vi "Game_Step.vi"(0 "State":T1={"Tick"=0, "Phase"=0, "PhaseTicks"=0, "Level"=1, "Room"=0, "X10"=0, "Y10"=0, "VY10"=0, "Mode"=0, "Facing"=0, "Run"=0, "Vert"=0, "StandY"=0, "EntryX10"=0, "EntryY10"=0, "EntryMode"=0, "Lives"=4, "Score"=0, "NextLife"=10000, "KeyR"=0, "KeyB"=0, "KeyY"=0, "Torch"=FALSE, "FloorPhase"=0, "Dead"=FALSE, "LevelStart"=FALSE, "Quit"=FALSE, "Sound"=0, "Seed"=12345, "DemoStep"=0, "Tiles"=[], "World"=[], "Enemies"=[], "Highscores"=[], "Name"=[0, 0, 0], "Cursor"=0}, 5 "Key":u16, 7 "Rooms":T2(array[cluster]), 11 "error in":errorcluster) -> (4 "State out":T1={"Tick"=0, "Phase"=0, "PhaseTicks"=0, "Level"=1, "Room"=0, "X10"=0, "Y10"=0, "VY10"=0, "Mode"=0, "Facing"=0, "Run"=0, "Vert"=0, "StandY"=0, "EntryX10"=0, "EntryY10"=0, "EntryMode"=0, "Lives"=4, "Score"=0, "NextLife"=10000, "KeyR"=0, "KeyB"=0, "KeyY"=0, "Torch"=FALSE, "FloorPhase"=0, "Dead"=FALSE, "LevelStart"=FALSE, "Quit"=FALSE, "Sound"=0, "Seed"=12345, "DemoStep"=0, "Tiles"=[], "World"=[], "Enemies"=[], "Highscores"=[], "Name"=[0, 0, 0], "Cursor"=0}, 15 "error out":errorcluster)   [LabVIEW 2020, in "GH_Engine.lvlib"]
doc: "One game tick, a state machine over the phases Title, Ready, Playing, Paused, Dying, Treasure, LevelDone, GameOver, Name, Demo. Title: card, short instructions, then the highscore table, then the demo; Enter starts, Esc quits. Ready: short pause with a message. Playing: Game_Play; a hit or a deadly fall starts Dying, the treasure room starts Treasure. Paused: Space, Enter or an arrow continues, Esc/P again ends the game (GameOver). Dying: one life less, then Ready at the arrival point or GameOver. Treasure: playing against the clock, then LevelDone and the next level. GameOver: then Name entry (arrows choose letters, Enter saves) when the score is good enough, else Title. Sound bits for the audio loop; music during Ready, Playing, Treasure. Keys: 0 None, 1 Up, 2 Down, 3 Left, 4 Right, 5 Quit, 6 Pause, 7 Start, 8 Jump, 9 Release, 10 ReleaseV, 11 ReleaseL, 12 ReleaseR, 13 Cheat."
uses:
  GH_Engine.lvlib
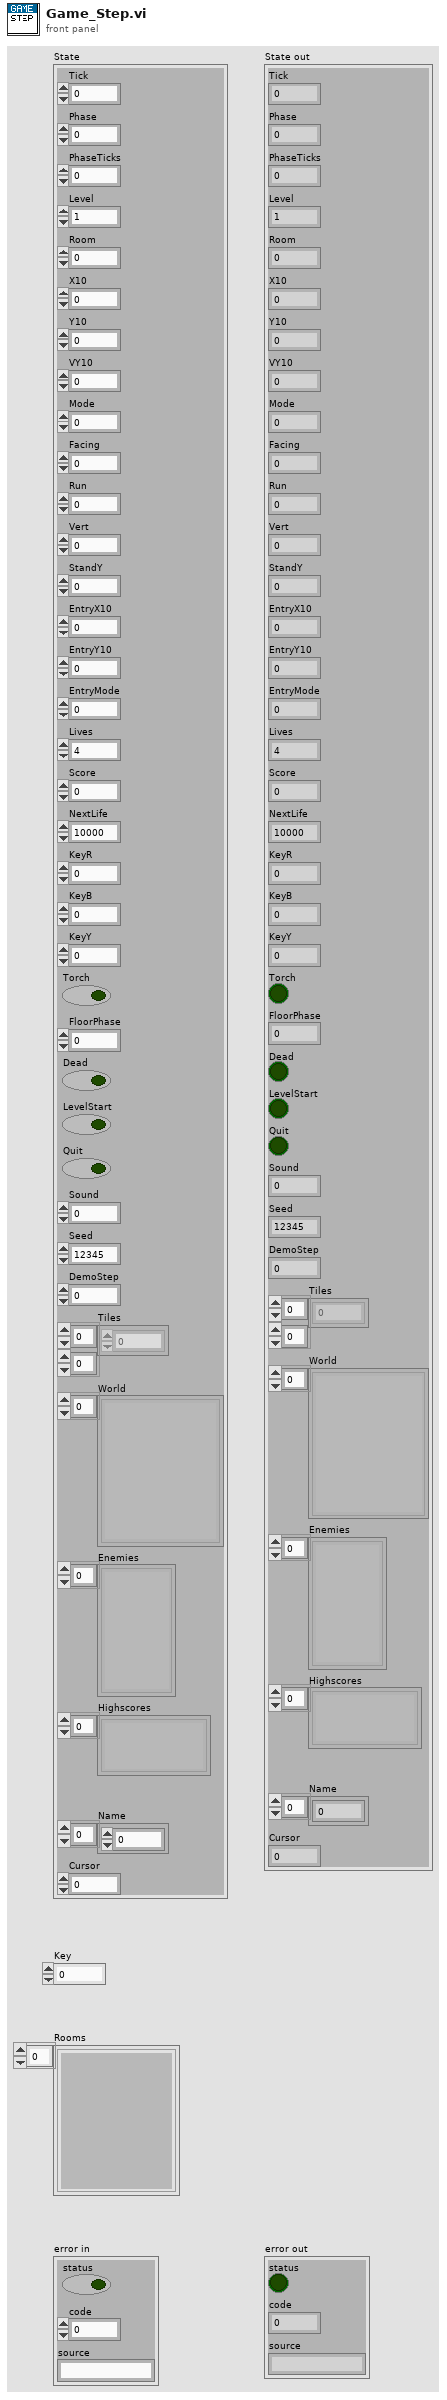
[diagram p1: front panel]
types:
  T1 = cluster{"Tick":u32, "Phase":i32, "PhaseTicks":i32, "Level":i32, "Room":i32, "X10":i32, "Y10":i32, "VY10":i32, "Mode":i32, "Facing":i32, "Run":i32, "Vert":i32, "StandY":i32, "EntryX10":i32, "EntryY10":i32, "EntryMode":i32, "Lives":i32, "Score":i32, "NextLife":i32, "KeyR":i32, "KeyB":i32, "KeyY":i32, "Torch":bool, "FloorPhase":i32, "Dead":bool, "LevelStart":bool, "Quit":bool, "Sound":i32, "Seed":u32, "DemoStep":i32, "Tiles":u8[][], "World":cluster{"ID":string, "Depth":i32, "Column":i32, "Tiles":u8[][]}[], "Enemies":cluster{"Kind":i32, "X10":i32, "Y10":i32, "Dir":i32, "Mode":i32}[], "Highscores":cluster{"Score":i32, "Name":string}[], "Name":i32[], "Cursor":i32}
  T2 = cluster{"ID":string, "Depth":i32, "Column":i32, "Tiles":u8[][]}[]
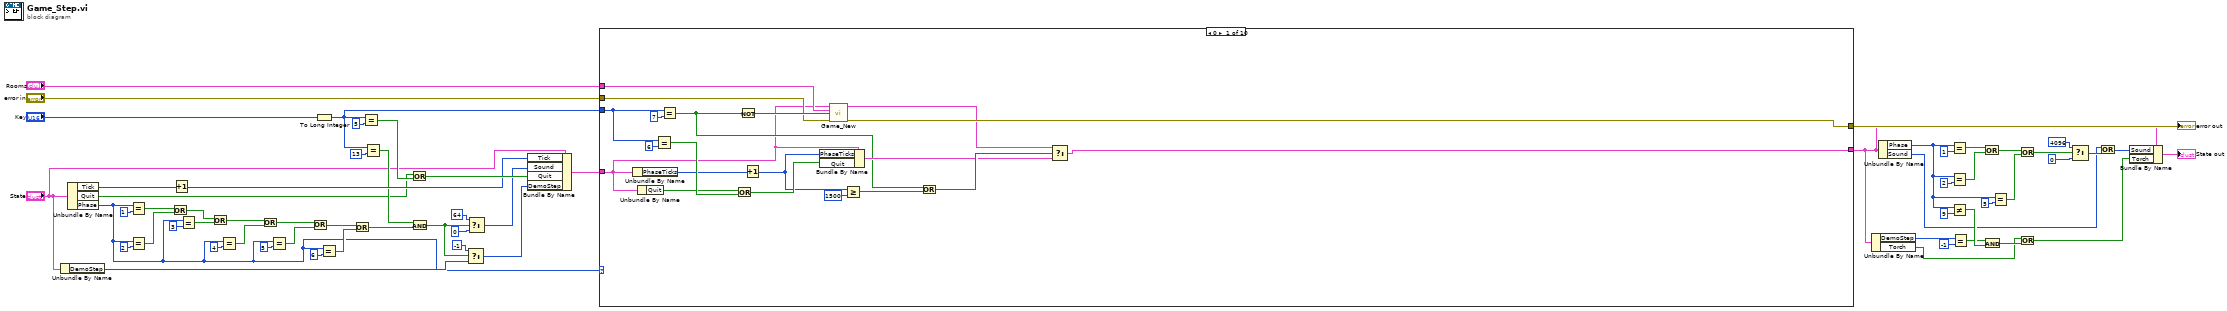
[diagram p0: block diagram]
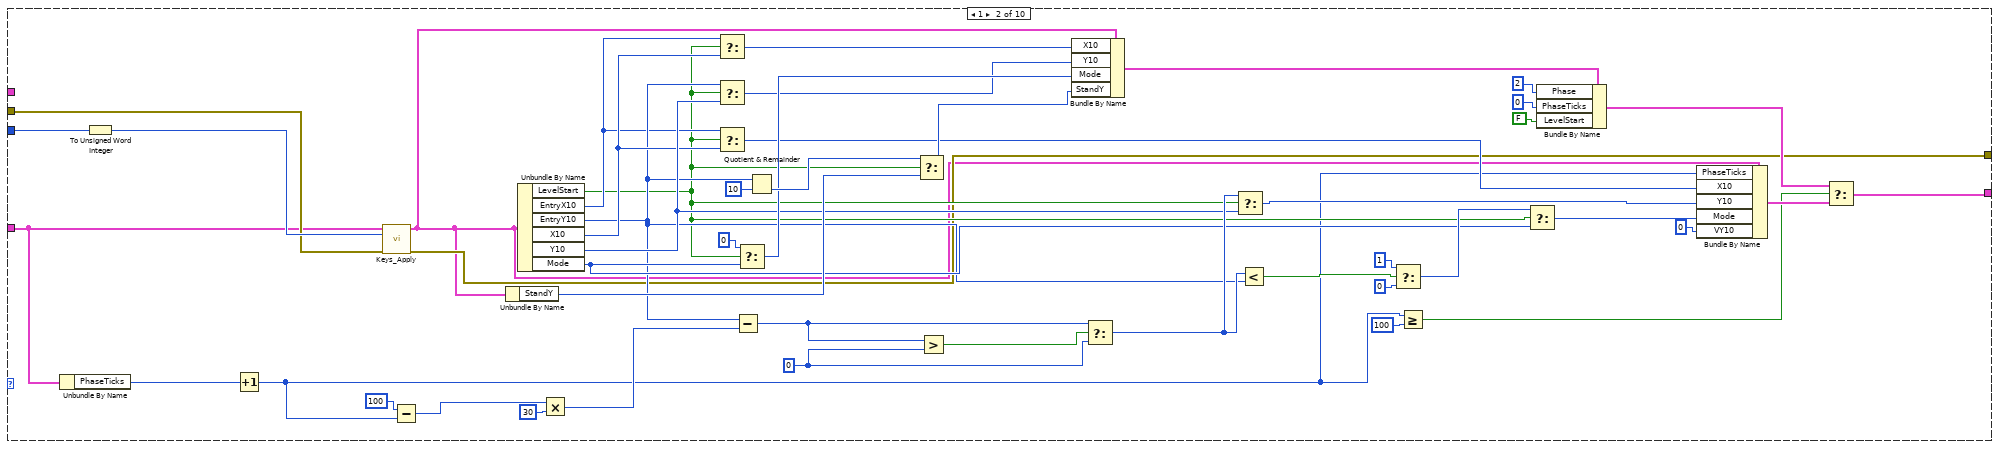
[diagram p2: hidden frame]
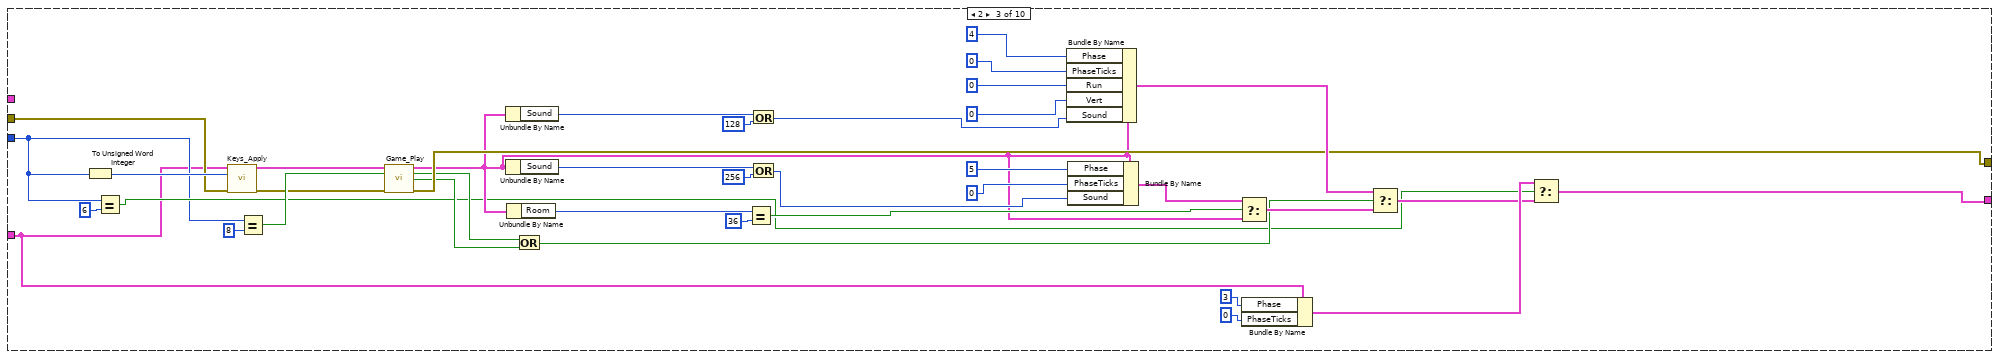
[diagram p3: hidden frame]
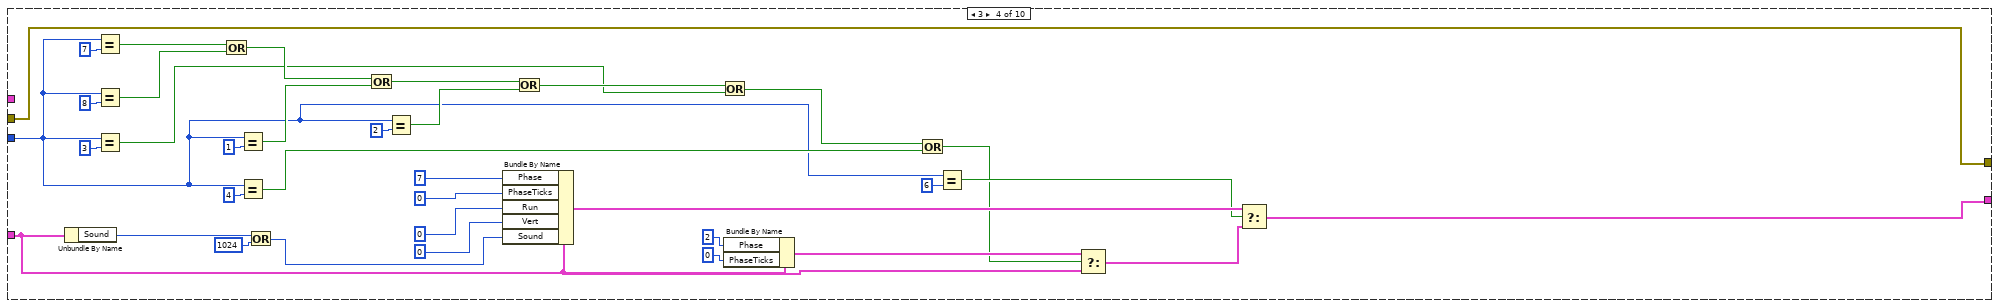
[diagram p4: hidden frame]
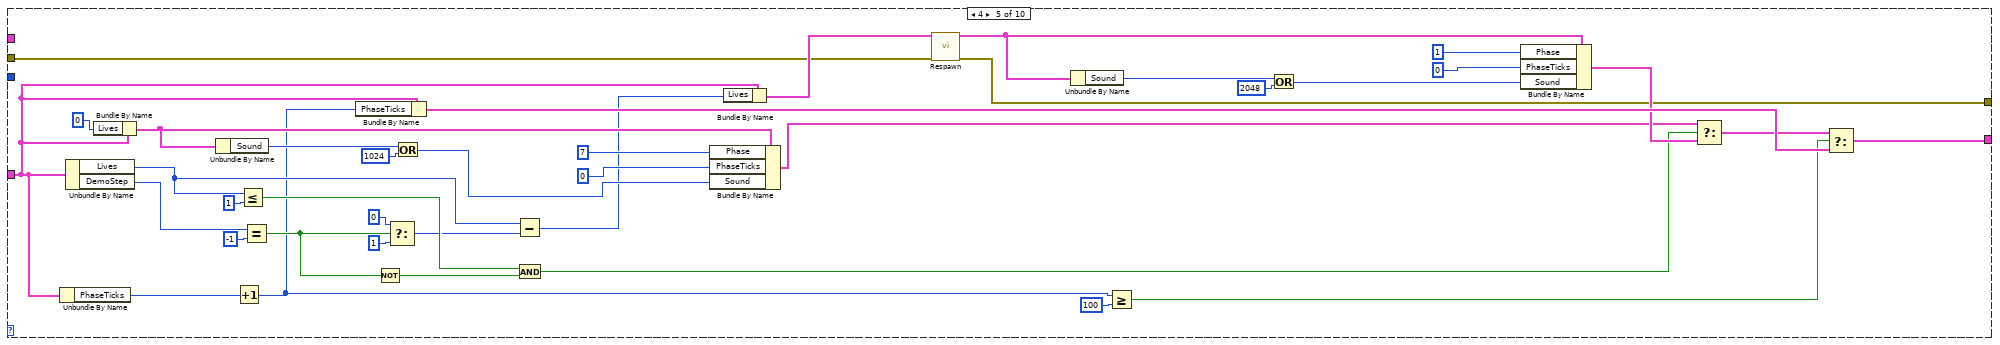
[diagram p5: hidden frame]
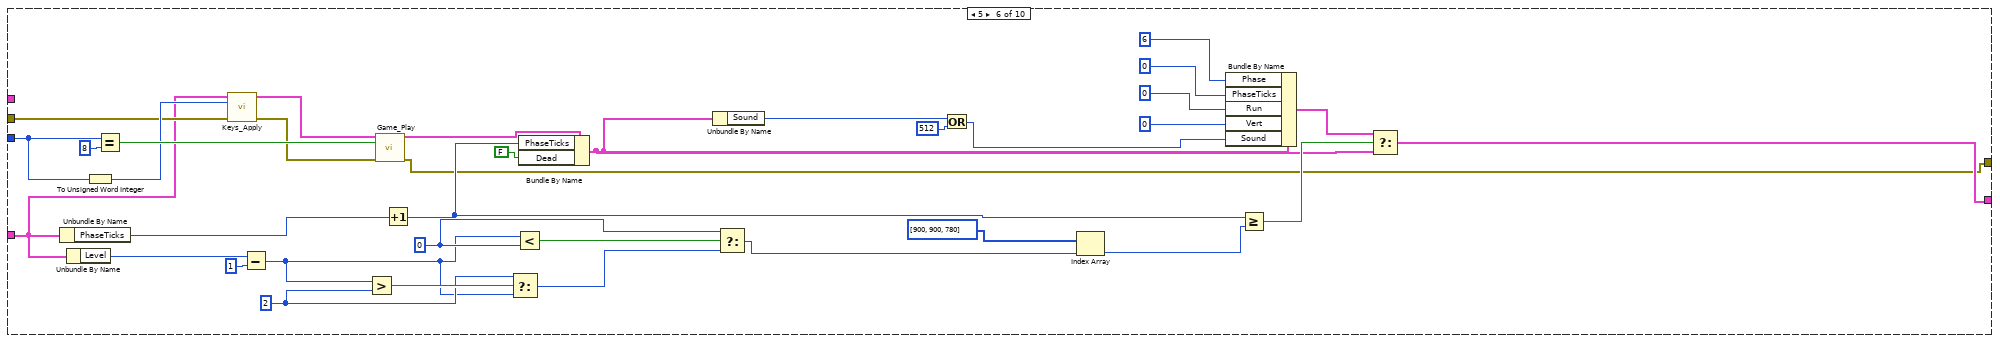
[diagram p6: hidden frame]
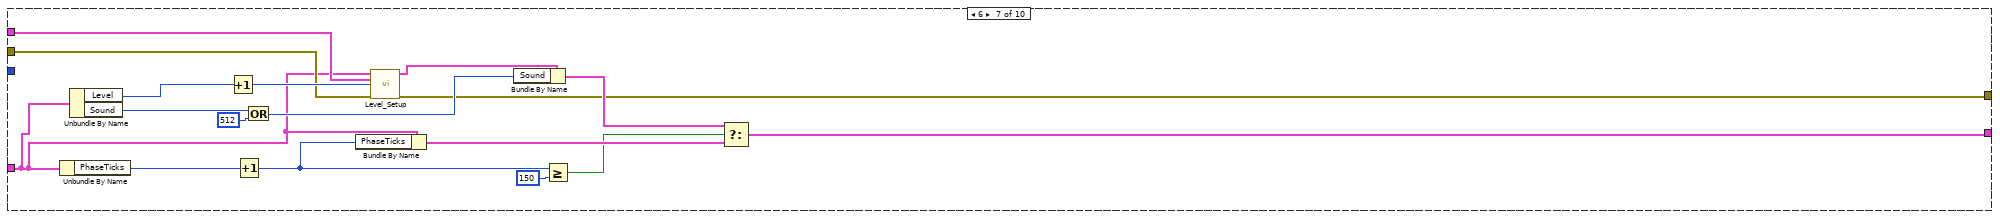
[diagram p7: hidden frame]
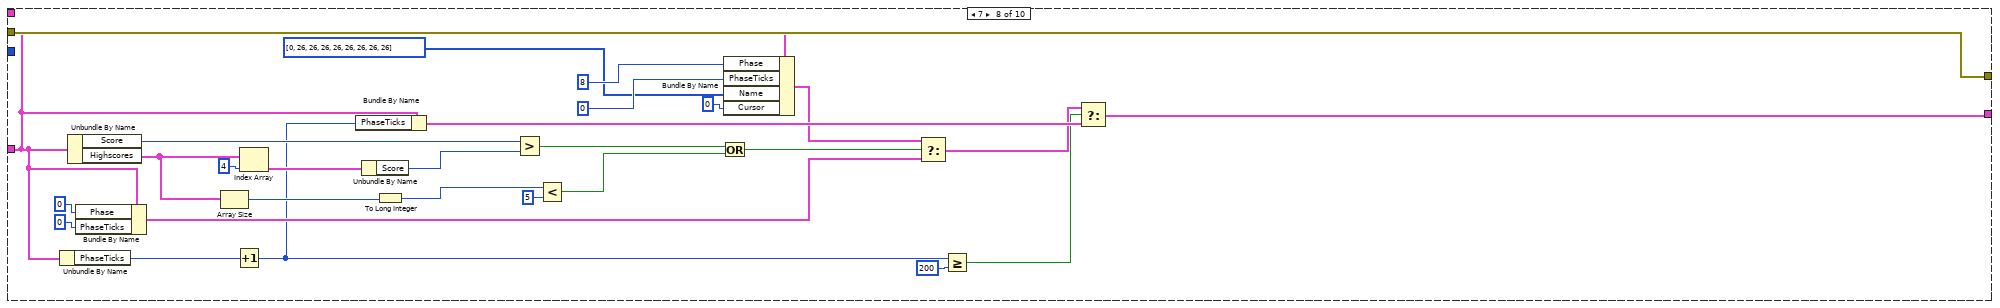
[diagram p8: hidden frame]
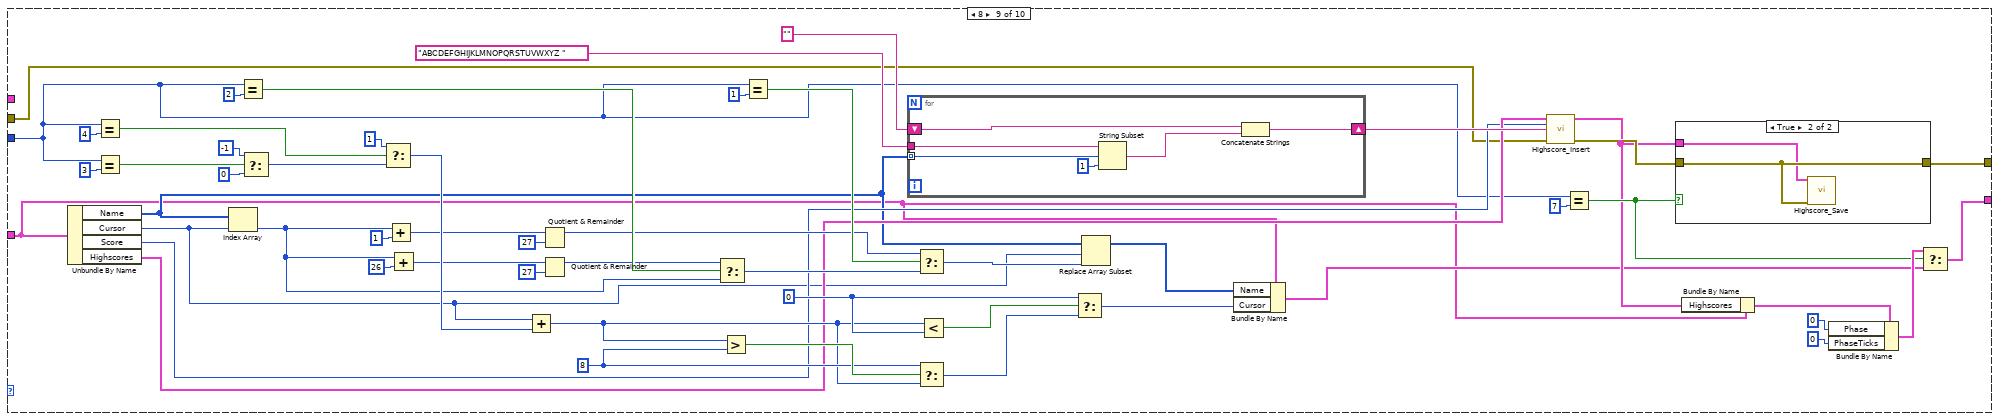
[diagram p9: hidden frame]
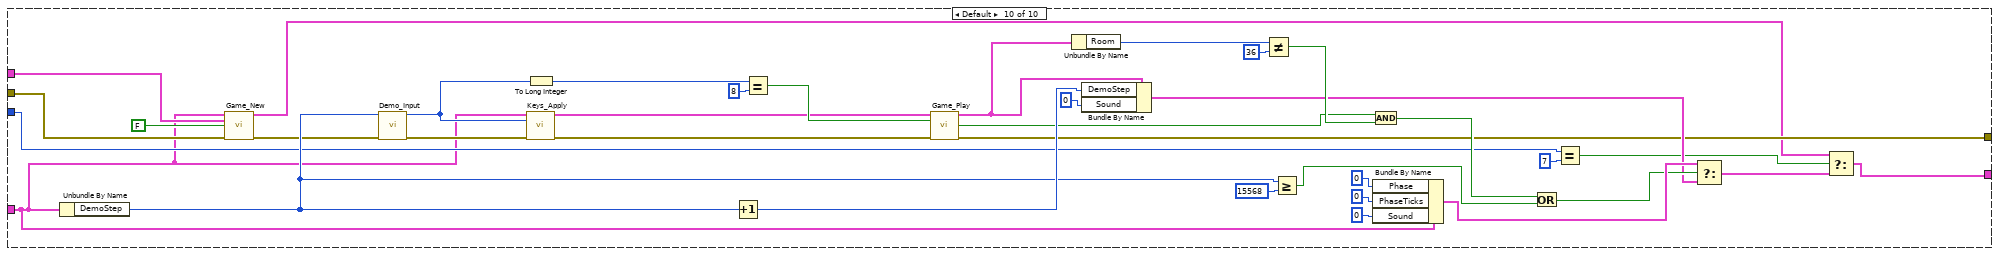
[diagram p11: hidden frame]
diagram:
  n1 = Unbundle By Name("State") -> ("DemoStep"=w29:i32)
  n2 = Unbundle By Name("State") -> ("Tick"=w6:u32, "Quit"=w7:bool, "Phase"=w8:i32)
  n3 = Equal?(x=w8, y=1) -> (x = y?=w10:bool)
  n4 = Equal?(x=w8, y=2) -> (x = y?=w12:bool)
  n5 = Or(x=w10, y=w12) -> (x .or. y?=w21:bool)
  n6 = Increment(x=w6) -> (x+1=w30:u32)
  n7 = Equal?(x=w8, y=3) -> (x = y?=w14:bool)
  n8 = Or(x=w21, y=w14) -> (x .or. y?=w22:bool)
  n9 = Equal?(x=w8, y=4) -> (x = y?=w16:bool)
  n10 = Or(x=w22, y=w16) -> (x .or. y?=w23:bool)
  n11 = Equal?(x=w8, y=5) -> (x = y?=w18:bool)
  n12 = Or(x=w23, y=w18) -> (x .or. y?=w24:bool)
  n13 = To Long Integer(number="Key") -> (32bit integer=w5:i32)
  n14 = Equal?(x=w8, y=6) -> (x = y?=w20:bool)
  n15 = Or(x=w24, y=w20) -> (x .or. y?=w25:bool)
  n16 = Equal?(x=w5, y=5) -> (x = y?=w35:bool)
  n17 = Equal?(x=w5, y=13) -> (x = y?=w27:bool)
  n18 = Or(x=w7, y=w35) -> (x .or. y?=w36:bool)
  n19 = And(x=w27, y=w25) -> (x .and. y?=w28:bool)
  n20 = Select(t=-1, s=w28, f=w29) -> (s? t:f=w38:i32)
  n21 = Select(t=64, s=w28, f=0) -> (s? t:f=w33:i32)
  n22 = Bundle By Name(cluster="State", "Tick"=w30, "Sound"=w33, "Quit"=w36, "DemoStep"=w38) -> (w39:T1)
  n23 = case shown="0" w8 {
    tunnel: "Rooms" -> [w67 _ _ _ _ _ w279 _ _ w387]
    tunnel: "error in" -> [w68 w87 w134 w172 w206 w245 w280 w296 w325 w388]
    tunnel: w5 -> [w66 w86 w133 w171 _ w244 _ _ w324 w386]
    tunnel: w39 -> [w65 w85 w132 w170 w205 w243 w278 w295 w323 w385]
    tunnel: [w77 w90 w145 w172 w219 w252 w287 w296 w370 w404] -> w41
    tunnel: [w84 w131 w169 w204 w242 w277 w294 w322 w375 w420] -> w40
    frame 0 {
      n24 = Unbundle By Name(w65) -> ("PhaseTicks"=w69:i32)
      n25 = Unbundle By Name(w65) -> ("Quit"=w78:bool)
      n26 = Equal?(x=w66, y=6) -> (x = y?=w80:bool)
      n27 = Equal?(x=w66, y=7) -> (x = y?=w72:bool)
      n28 = Or(x=w78, y=w80) -> (x .or. y?=w81:bool)
      n29 = Not(x=w72) -> (.not. x?=w75:bool)
      n30 = Increment(x=w69) -> (x+1=w70:i32)
      n31 = Bundle By Name(cluster=w65, "PhaseTicks"=w70, "Quit"=w81) -> (w82:T1)
      n32 = call "Game_New.vi"("State"=w65, "Rooms"=w67, "Demo"=w75, "error in"=w68) -> ("State out"=w76:T1, "error out"=w77:errorcluster)  [unwired: 10 in]
      n33 = Greater Or Equal?(x=w70, y=1500) -> (x >= y?=w74:bool)
      n34 = Or(x=w72, y=w74) -> (x .or. y?=w83:bool)
      n35 = Select(t=w76, s=w83, f=w82) -> (s? t:f=w84:T1)
    }
    frame 1 {
      w106 = 0
      n36 = Unbundle By Name(w85) -> ("PhaseTicks"=w91:i32)
      n37 = To Unsigned Word Integer(number=w86) -> (unsigned 16bit integer=w88:u16)
      n38 = Increment(x=w91) -> (x+1=w92:i32)
      n39 = call "Keys_Apply.vi"("State"=w85, "Key"=w88, "error in"=w87) -> ("State out"=w89:T1, "error out"=w90:errorcluster)  [unwired: 11 in]
      n40 = Subtract(x=100, y=w92) -> (x-y=w102:i32)
      n41 = Unbundle By Name(w89) -> ("StandY"=w124:i32)
      n42 = Unbundle By Name(w89) -> ("LevelStart"=w95:bool, "EntryX10"=w96:i32, "EntryY10"=w97:i32, "X10"=w98:i32, "Y10"=w99:i32, "Mode"=w100:i32)
      n43 = Multiply(x=w102, y=30) -> (x*y=w104:i32)
      n44 = Select(t=w96, s=w95, f=w98) -> (s? t:f=w118:i32)
      n45 = Select(t=w97, s=w95, f=w99) -> (s? t:f=w119:i32)
      n46 = Select(t=w96, s=w95, f=w98) -> (s? t:f=w109:i32)
      n47 = Subtract(x=w97, y=w104) -> (x-y=w105:i32)
      n48 = Select(t=0, s=w95, f=w100) -> (s? t:f=w121:i32)
      n49 = Quotient & Remainder(x=w97, y=10) -> (floor(x/y)=w123:i32)  [unwired: 1 out]
      n50 = Select(t=w123, s=w95, f=w124) -> (s? t:f=w125:i32)
      n51 = Greater?(x=w105, y=w106) -> (0:w107:bool)
      n52 = Bundle By Name(cluster=w89, "X10"=w118, "Y10"=w119, "Mode"=w121, "StandY"=w125) -> (w126:T1)
      n53 = Select(t=w105, s=w107, f=w106) -> (s? t:f=w108:i32)
      n54 = Select(t=w108, s=w95, f=w99) -> (s? t:f=w110:i32)
      n55 = Less?(x=w108, y=w97) -> (x < y?=w111:bool)
      n56 = Select(t=1, s=w111, f=0) -> (s? t:f=w114:i32)
      n57 = Greater Or Equal?(x=w92, y=100) -> (x >= y?=w94:bool)
      n58 = Select(t=w114, s=w95, f=w100) -> (s? t:f=w115:i32)
      n59 = Bundle By Name(cluster=w126, "Phase"=2, "PhaseTicks"=0, "LevelStart"=FALSE) -> (w130:T1)
      n60 = Bundle By Name(cluster=w89, "PhaseTicks"=w92, "X10"=w109, "Y10"=w110, "Mode"=w115, "VY10"=0) -> (w117:T1)
      n61 = Select(t=w130, s=w94, f=w117) -> (s? t:f=w131:T1)
    }
    frame 2 {
      n62 = To Unsigned Word Integer(number=w133) -> (unsigned 16bit integer=w137:u16)
      n63 = Equal?(x=w133, y=6) -> (x = y?=w136:bool)
      n64 = call "Keys_Apply.vi"("State"=w132, "Key"=w137, "error in"=w134) -> ("State out"=w138:T1, "error out"=w139:errorcluster)  [unwired: 11 in]
      n65 = Equal?(x=w133, y=8) -> (x = y?=w141:bool)
      n66 = call "Game_Play.vi"("State"=w138, "Jump"=w141, "error in"=w139) -> ("State out"=w142:T1, "Hit"=w143:bool, "Died"=w144:bool, "error out"=w145:errorcluster)  [unwired: 9 in]
      n67 = Unbundle By Name(w142) -> ("Sound"=w151:i32)
      n68 = Unbundle By Name(w142) -> ("Sound"=w157:i32)
      n69 = Unbundle By Name(w142) -> ("Room"=w146:i32)
      n70 = Or(x=w143, y=w144) -> (x .or. y?=w161:bool)
      n71 = Equal?(x=w146, y=36) -> (x = y?=w163:bool)
      n72 = Or(x=w151, y=128) -> (x .or. y?=w153:i32)
      n73 = Or(x=w157, y=256) -> (x .or. y?=w159:i32)
      n74 = Bundle By Name(cluster=w142, "Phase"=4, "PhaseTicks"=0, "Run"=0, "Vert"=0, "Sound"=w153) -> (w154:T1)
      n75 = Bundle By Name(cluster=w142, "Phase"=5, "PhaseTicks"=0, "Sound"=w159) -> (w160:T1)
      n76 = Select(t=w160, s=w163, f=w142) -> (s? t:f=w164:T1)
      n77 = Bundle By Name(cluster=w132, "Phase"=3, "PhaseTicks"=0) -> (w168:T1)
      n78 = Select(t=w154, s=w161, f=w164) -> (s? t:f=w165:T1)
      n79 = Select(t=w168, s=w136, f=w165) -> (s? t:f=w169:T1)
    }
    frame 3 {
      n80 = Unbundle By Name(w170) -> ("Sound"=w196:i32)
      n81 = Equal?(x=w171, y=7) -> (x = y?=w174:bool)
      n82 = Equal?(x=w171, y=8) -> (x = y?=w176:bool)
      n83 = Equal?(x=w171, y=3) -> (x = y?=w182:bool)
      n84 = Or(x=w174, y=w176) -> (x .or. y?=w185:bool)
      n85 = Equal?(x=w171, y=1) -> (x = y?=w178:bool)
      n86 = Equal?(x=w171, y=4) -> (x = y?=w184:bool)
      n87 = Or(x=w196, y=1024) -> (x .or. y?=w198:i32)
      n88 = Or(x=w185, y=w178) -> (x .or. y?=w186:bool)
      n89 = Equal?(x=w171, y=2) -> (x = y?=w180:bool)
      n90 = Bundle By Name(cluster=w170, "Phase"=7, "PhaseTicks"=0, "Run"=0, "Vert"=0, "Sound"=w198) -> (w199:T1)
      n91 = Or(x=w186, y=w180) -> (x .or. y?=w187:bool)
      n92 = Or(x=w187, y=w182) -> (x .or. y?=w188:bool)
      n93 = Bundle By Name(cluster=w170, "Phase"=2, "PhaseTicks"=0) -> (w202:T1)
      n94 = Or(x=w188, y=w184) -> (x .or. y?=w189:bool)
      n95 = Equal?(x=w171, y=6) -> (x = y?=w191:bool)
      n96 = Select(t=w202, s=w189, f=w170) -> (s? t:f=w203:T1)
      n97 = Select(t=w199, s=w191, f=w203) -> (s? t:f=w204:T1)
    }
    frame 4 {
      n98 = Unbundle By Name(w205) -> ("PhaseTicks"=w207:i32)
      n99 = Unbundle By Name(w205) -> ("Lives"=w209:i32, "DemoStep"=w210:i32)
      n100 = Bundle By Name(cluster=w205, "Lives"=0) -> (w227:T1)
      n101 = Unbundle By Name(w227) -> ("Sound"=w230:i32)
      n102 = Increment(x=w207) -> (x+1=w208:i32)
      n103 = Less Or Equal?(x=w209, y=1) -> (x <= y?=w223:bool)
      n104 = Equal?(x=w210, y=-1) -> (x = y?=w212:bool)
      n105 = Bundle By Name(cluster=w205, "PhaseTicks"=w208) -> (w241:T1)
      n106 = Not(x=w212) -> (.not. x?=w224:bool)
      n107 = Select(t=0, s=w212, f=1) -> (s? t:f=w215:i32)
      n108 = Or(x=w230, y=1024) -> (x .or. y?=w232:i32)
      n109 = Subtract(x=w209, y=w215) -> (x-y=w216:i32)
      n110 = And(x=w223, y=w224) -> (x .and. y?=w225:bool)
      n111 = Bundle By Name(cluster=w227, "Phase"=7, "PhaseTicks"=0, "Sound"=w232) -> (w233:T1)
      n112 = Bundle By Name(cluster=w205, "Lives"=w216) -> (w217:T1)
      n113 = call "Respawn.vi"("State"=w217, "error in"=w206) -> ("State out"=w218:T1, "error out"=w219:errorcluster)  [unwired: 12 in]
      n114 = Unbundle By Name(w218) -> ("Sound"=w236:i32)
      n115 = Greater Or Equal?(x=w208, y=100) -> (x >= y?=w221:bool)
      n116 = Or(x=w236, y=2048) -> (x .or. y?=w238:i32)
      n117 = Bundle By Name(cluster=w218, "Phase"=1, "PhaseTicks"=0, "Sound"=w238) -> (w239:T1)
      n118 = Select(t=w233, s=w225, f=w239) -> (s? t:f=w240:T1)
      n119 = Select(t=w240, s=w221, f=w241) -> (s? t:f=w242:T1)
    }
    frame 5 {
      w260 = 2
      w259 = 0
      n120 = Unbundle By Name(w243) -> ("PhaseTicks"=w253:i32)
      n121 = Unbundle By Name(w243) -> ("Level"=w255:i32)
      n122 = To Unsigned Word Integer(number=w244) -> (unsigned 16bit integer=w246:u16)
      n123 = Equal?(x=w244, y=8) -> (x = y?=w250:bool)
      n124 = call "Keys_Apply.vi"("State"=w243, "Key"=w246, "error in"=w245) -> ("State out"=w247:T1, "error out"=w248:errorcluster)  [unwired: 11 in]
      n125 = Subtract(x=w255, y=1) -> (x-y=w258:i32)
      n126 = Greater?(x=w258, y=w260) -> (0:w262:bool)
      n127 = call "Game_Play.vi"("State"=w247, "Jump"=w250, "error in"=w248) -> ("State out"=w251:T1, "error out"=w252:errorcluster)  [unwired: 9 in, 2 out]
      n128 = Increment(x=w253) -> (x+1=w254:i32)
      n129 = Select(t=w260, s=w262, f=w258) -> (s? t:f=w263:i32)
      n130 = Less?(x=w258, y=w259) -> (x < y?=w261:bool)
      n131 = Bundle By Name(cluster=w251, "PhaseTicks"=w254, "Dead"=FALSE) -> (w267:T1)
      n132 = Unbundle By Name(w267) -> ("Sound"=w272:i32)
      n133 = Select(t=w259, s=w261, f=w263) -> (s? t:f=w264:i32)
      n134 = Or(x=w272, y=512) -> (x .or. y?=w274:i32)
      n135 = Index Array(array=i32[] [900, 900, 780] ("Treasure time"), index=w264) -> (element=w265:i32)
      n136 = Bundle By Name(cluster=w267, "Phase"=6, "PhaseTicks"=0, "Run"=0, "Vert"=0, "Sound"=w274) -> (w275:T1)
      n137 = Greater Or Equal?(x=w254, y=w265) -> (x >= y?=w276:bool)
      n138 = Select(t=w275, s=w276, f=w267) -> (s? t:f=w277:T1)
    }
    frame 6 {
      n139 = Unbundle By Name(w278) -> ("PhaseTicks"=w281:i32)
      n140 = Unbundle By Name(w278) -> ("Level"=w283:i32, "Sound"=w284:i32)
      n141 = Increment(x=w283) -> (x+1=w285:i32)
      n142 = Increment(x=w281) -> (x+1=w282:i32)
      n143 = Or(x=w284, y=512) -> (x .or. y?=w289:i32)
      n144 = Bundle By Name(cluster=w278, "PhaseTicks"=w282) -> (w293:T1)
      n145 = call "Level_Setup.vi"("State"=w278, "Rooms"=w279, "Level"=w285, "error in"=w280) -> ("State out"=w286:T1, "error out"=w287:errorcluster)  [unwired: 10 in]
      n146 = Bundle By Name(cluster=w286, "Sound"=w289) -> (w290:T1)
      n147 = Greater Or Equal?(x=w282, y=150) -> (x >= y?=w292:bool)
      n148 = Select(t=w290, s=w292, f=w293) -> (s? t:f=w294:T1)
    }
    frame 7 {
      n149 = Unbundle By Name(w295) -> ("PhaseTicks"=w297:i32)
      n150 = Unbundle By Name(w295) -> ("Score"=w299:i32, "Highscores"=w300:cluster{"Score":i32, "Name":string}[])
      n151 = Bundle By Name(cluster=w295, "Phase"=0, "PhaseTicks"=0) -> (w317:T1)
      n152 = Array Size(array=w300) -> (size(s)=w305:i32)
      n153 = Increment(x=w297) -> (x+1=w298:i32)
      n154 = Index Array(array=w300, index=4) -> (element=w302:cluster{"Score":i32, "Name":string})
      n155 = Bundle By Name(cluster=w295, "PhaseTicks"=w298) -> (w321:T1)
      n156 = Unbundle By Name(w302) -> ("Score"=w303:i32)
      n157 = To Long Integer(number=w305) -> (32bit integer=w306:i32)
      n158 = Greater?(x=w299, y=w303) -> (0:w304:bool)
      n159 = Less?(x=w306, y=5) -> (x < y?=w308:bool)
      n160 = Or(x=w304, y=w308) -> (x .or. y?=w309:bool)
      n161 = Bundle By Name(cluster=w295, "Phase"=8, "PhaseTicks"=0, "Name"=i32[] [0, 26, 26, 26, 26, 26, 26, 26, 26], "Cursor"=0) -> (w314:T1)
      n162 = Select(t=w314, s=w309, f=w317) -> (s? t:f=w320:T1)
      n163 = Greater Or Equal?(x=w298, y=200) -> (x >= y?=w319:bool)
      n164 = Select(t=w320, s=w319, f=w321) -> (s? t:f=w322:T1)
    }
    frame 8 {
      w357 = 8
      w356 = 0
      n165 = Unbundle By Name(w323) -> ("Name"=w326:i32[], "Cursor"=w327:i32, "Score"=w328:i32, "Highscores"=w329:cluster{"Score":i32, "Name":string}[])
      n166 = Equal?(x=w324, y=4) -> (x = y?=w347:bool)
      n167 = Equal?(x=w324, y=3) -> (x = y?=w350:bool)
      n168 = Index Array(array=w326, index=w327) -> (element=w330:i32)
      n169 = Equal?(x=w324, y=2) -> (x = y?=w342:bool)
      n170 = Select(t=-1, s=w350, f=0) -> (s? t:f=w353:i32)
      n171 = Select(t=1, s=w347, f=w353) -> (s? t:f=w354:i32)
      n172 = Add(x=w330, y=1) -> (x+y=w332:i32)
      n173 = Add(x=w330, y=26) -> (x+y=w336:i32)
      n174 = Add(x=w327, y=w354) -> (x+y=w355:i32)
      n175 = Quotient & Remainder(x=w332, y=27) -> (x-y*floor(x/y)=w334:i32)  [unwired: 1 out]
      n176 = Quotient & Remainder(x=w336, y=27) -> (x-y*floor(x/y)=w338:i32)  [unwired: 1 out]
      n177 = Select(t=w338, s=w342, f=w330) -> (s? t:f=w343:i32)
      n178 = Greater?(x=w355, y=w357) -> (0:w359:bool)
      n179 = Equal?(x=w324, y=1) -> (x = y?=w340:bool)
      n180 = for {
        tunnel: "ABCDEFGHIJKLMNOPQRSTUVWXYZ " -> [w380]
        shift-right: [w382] -> w365
        shift-left: "" -> [w381]
        tunnel: w326 -> [w379] mode=indexing
        n181 = String Subset(string=w380, offset (0)=w379, length (rest)=1) -> (substring=w384:string)
        n182 = Concatenate Strings(w381, w384) -> (w382:string)
      }
      n183 = Select(t=w334, s=w340, f=w343) -> (s? t:f=w344:i32)
      n184 = Select(t=w357, s=w359, f=w355) -> (s? t:f=w360:i32)
      n185 = Less?(x=w355, y=w356) -> (x < y?=w358:bool)
      n186 = Select(t=w356, s=w358, f=w360) -> (s? t:f=w361:i32)
      n187 = Replace Array Subset(array=w326, new element=w344, index=w327) -> (w345:i32[])
      n188 = Bundle By Name(cluster=w323, "Name"=w345, "Cursor"=w361) -> (w362:T1)
      n189 = call "Highscore_Insert.vi"("Table"=w329, "Score"=w328, "Name"=w365, "error in"=w325) -> ("Table out"=w366:cluster{"Score":i32, "Name":string}[], "error out"=w367:errorcluster)  [unwired: 10 in]
      n190 = Equal?(x=w324, y=7) -> (x = y?=w369:bool)
      n191 = case shown="True" w369 {
        tunnel: w366 -> [_ w377]
        tunnel: w367 -> [w376 w378]
        tunnel: [w376 w378] -> w370
        frame False {
        }
        frame True {
          n192 = call "Highscore_Save.vi"("Table"=w377, "error in"=w378) -> ()  [unwired: 13 in, 1 out]
        }
      }
      n193 = Bundle By Name(cluster=w323, "Highscores"=w366) -> (w371:T1)
      n194 = Bundle By Name(cluster=w371, "Phase"=0, "PhaseTicks"=0) -> (w374:T1)
      n195 = Select(t=w374, s=w369, f=w362) -> (s? t:f=w375:T1)
    }
    frame Default {
      n196 = Unbundle By Name(w385) -> ("DemoStep"=w394:i32)
      n197 = call "Game_New.vi"("State"=w385, "Rooms"=w387, "Demo"=FALSE, "error in"=w388) -> ("State out"=w392:T1, "error out"=w393:errorcluster)  [unwired: 10 in]
      n198 = call "Demo_Input.vi"("Step"=w394, "error in"=w393) -> ("Key"=w395:u16, "error out"=w396:errorcluster)  [unwired: 12 in]
      n199 = call "Keys_Apply.vi"("State"=w385, "Key"=w395, "error in"=w396) -> ("State out"=w397:T1, "error out"=w398:errorcluster)  [unwired: 11 in]
      n200 = To Long Integer(number=w395) -> (32bit integer=w399:i32)
      n201 = Increment(x=w394) -> (x+1=w406:i32)
      n202 = Equal?(x=w399, y=8) -> (x = y?=w401:bool)
      n203 = call "Game_Play.vi"("State"=w397, "Jump"=w401, "error in"=w398) -> ("State out"=w402:T1, "Died"=w403:bool, "error out"=w404:errorcluster)  [unwired: 9 in, 1 out]
      n204 = Unbundle By Name(w402) -> ("Room"=w405:i32)
      n205 = Bundle By Name(cluster=w402, "DemoStep"=w406, "Sound"=0) -> (w408:T1)
      n206 = Not Equal?(x=w405, y=36) -> (x != y?=w410:bool)
      n207 = Greater Or Equal?(x=w394, y=15568) -> (x >= y?=w413:bool)
      n208 = And(x=w403, y=w410) -> (x .and. y?=w411:bool)
      n209 = Bundle By Name(cluster=w385, "Phase"=0, "PhaseTicks"=0, "Sound"=0) -> (w418:T1)
      n210 = Or(x=w411, y=w413) -> (x .or. y?=w414:bool)
      n211 = Equal?(x=w386, y=7) -> (x = y?=w390:bool)
      n212 = Select(t=w418, s=w414, f=w408) -> (s? t:f=w419:T1)
      n213 = Select(t=w392, s=w390, f=w419) -> (s? t:f=w420:T1)
    }
  }
  "error out" <- w41
  n214 = Unbundle By Name(w40) -> ("DemoStep"=w52:i32, "Torch"=w53:bool)
  n215 = Unbundle By Name(w40) -> ("Phase"=w42:i32, "Sound"=w43:i32)
  n216 = Equal?(x=w42, y=1) -> (x = y?=w45:bool)
  n217 = Equal?(x=w42, y=2) -> (x = y?=w47:bool)
  n218 = Not Equal?(x=w42, y=9) -> (x != y?=w57:bool)
  n219 = Equal?(x=w52, y=-1) -> (x = y?=w55:bool)
  n220 = Or(x=w45, y=w47) -> (x .or. y?=w50:bool)
  n221 = And(x=w55, y=w57) -> (x .and. y?=w58:bool)
  n222 = Equal?(x=w42, y=5) -> (x = y?=w49:bool)
  n223 = Or(x=w50, y=w49) -> (x .or. y?=w51:bool)
  n224 = Or(x=w53, y=w58) -> (x .or. y?=w63:bool)
  n225 = Select(t=4096, s=w51, f=0) -> (s? t:f=w61:i32)
  n226 = Or(x=w43, y=w61) -> (x .or. y?=w62:i32)
  n227 = Bundle By Name(cluster=w40, "Sound"=w62, "Torch"=w63) -> (→"State out":T1)
